vi "Unlock ECU.vi"(8 "error in (no error)":errorcluster, 11 "Node Ptr":T2 format="%.0x") -> (0 "error out":errorcluster)   [LabVIEW 2024, in "Diagnostics Addon System Explorer.lvlib"]
uses:
  Diagnostics Addon System Explorer.lvlib
  Addon Shared/Types/Security.Type.ctl
  <vilib>/NI VeriStand/Custom Device API/Custom Device Item Ref.ctl
  Types/FG.Action.ctl
  Addon Shared/Types/Settings.Channel.ctl
  <vilib>/NI VeriStand/Custom Device API/Custom Device Channel.ctl
  <vilib>/NI VeriStand/Custom Device API/Custom Device Channel Type.ctl
  SubVIs/FileDependency.Create.vi
  Addon Shared/SubVIs/Constants.vi
  <vilib>/NI VeriStand/Custom Device API/NI VeriStand - Get Item Property.vi
  <vilib>/NI VeriStand/Custom Device API/Get Item Property (U32).vi
  <vilib>/NI VeriStand/Custom Device API/Get Item Property (Path).vi
  SubVIs/FileDependency.Get.Target Path.vi
  <vilib>/NI VeriStand/Custom Device API/Get Item Property (Variant).vi
  <vilib>/NI VeriStand/Custom Device API/Get Item Property (String).vi
  <vilib>/NI VeriStand/Custom Device API/Get Item Property (I32).vi
  <vilib>/NI/NI VeriStand Advanced SysDef API/SysDef API/SysDef.Property.Remove.vi
  <vilib>/NI/NI VeriStand Advanced SysDef API/SysDef API/SysDef.Property.Set.vi
  <vilib>/NI/NI VeriStand Advanced SysDef API/_SubVIs/SysDef.Property.Set.Path.vi
  <vilib>/Utility/MD5Checksum.llb/MD5Checksum File.vi
  <vilib>/NI/NI VeriStand Advanced SysDef API/_SubVIs/SysDef.Property.Set.DependentFile.vi
  <vilib>/NI/NI VeriStand Advanced SysDef API/_SubVIs/SysDef.Property.Set.U32.vi
  <vilib>/NI/NI VeriStand Advanced SysDef API/_SubVIs/SysDef.Property.Set.Variant.vi
  <vilib>/NI/NI VeriStand Advanced SysDef API/_SubVIs/SysDef.Property.Set.String.vi
  <vilib>/NI/NI VeriStand Advanced SysDef API/_SubVIs/SysDef.Property.Set.I32.vi
  <vilib>/NI VeriStand/Custom Device Tools/Custom Device Utility Library/NI VeriStand - Search for Item by GUID.vi
  <vilib>/NI VeriStand/Custom Device API/Custom Device API.lvlib
  Addon Shared/Diagnostics Addon Shared.lvlib
  <vilib>/NI VeriStand/Custom Device Tools/Custom Device Utility Library/Custom Device Utility Library.lvlib
panel:
  in  "Host IP Address":string
  in  "Max Key Length":u32
  in  "Optional Parameter":i8 format="%.0x"
  in  "ECU Variant":i8 format="%.0x"
  in  "Access Mode":u32 format="%.0x"
  in  "Seed Key Path":path caption="Seed Key Path (.DLL or .SO)"
  in  "Type":T1
  in  "Master Key":string
  in  "Header":cluster{"Section Name":string}={"Section Name"="Security Settings"}
  in  "SHDocVw.IWebBrowser":refnum<k7>(container)
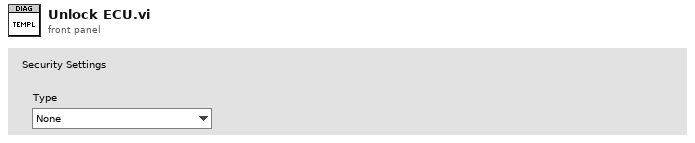
[diagram p1: front panel]
types:
  T1 = typedef "Diagnostics Addon Shared.lvlib/Security.Type.ctl" = enum16{"None", "SeedKey DLL", "MasterKey (Channel)", "MasterKey (Static)", "SeedKey DLL (Windows)"}
  T2 = typedef "Custom Device API.lvlib/Custom Device Item Ref.ctl" = u64
  T3 = typedef "Diagnostics Addon System Explorer.lvlib/FG.Action.ctl" = enum16{"Get", "Set"}
  T4 = typedef "Custom Device API.lvlib/Custom Device Item Info.ctl" = cluster{"Name":string, "Is Channel":bool, "GUID":string, "Is Waveform":bool}
  T5 = typedef "Diagnostics Addon Shared.lvlib/Security.ctl" = cluster{"Type":T1, "Source DLL Path":path, "Target DLL Path":path, "Security Level":u32, "Static Master Key":string, "Max Key Length":u32, "Host IP Address":string, "ECU  Variant":i8, "Optional Parameter":i8}
  T6 = typedef "Custom Device API.lvlib/Custom Device Commands.ctl" = enum16{"Default", "Item renamed", "Shutdown", "Dynamic button pressed"}
  T7 = typedef "Diagnostics Addon Shared.lvlib/Settings.Channel.ctl" = cluster{"Name":string, "Description":string, "Channel":T8}
  T8 = typedef "Custom Device API.lvlib/Custom Device Channel.ctl" = cluster{"Type":T9, "Units":string, "Default Value":dbl, "Faultable":bool, "Scalable":bool}
  T9 = typedef "Custom Device API.lvlib/Custom Device Channel Type.ctl" = enum16{"Input", "Output"}
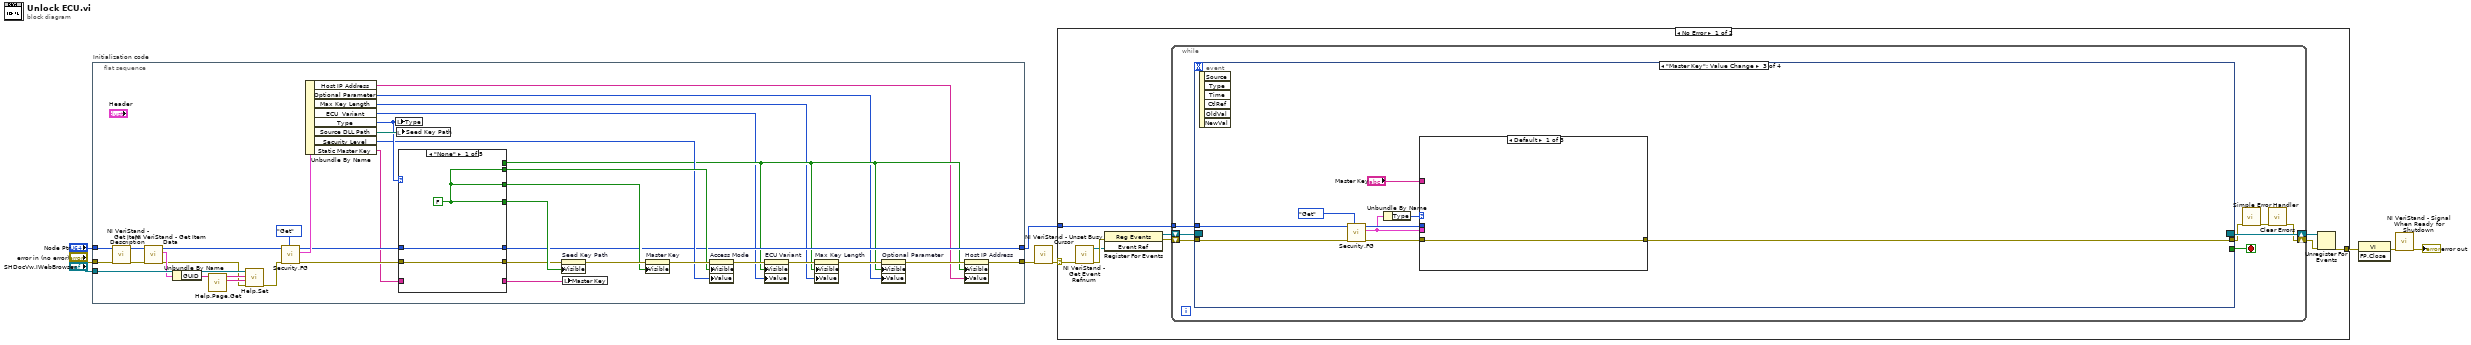
[diagram p0: block diagram]
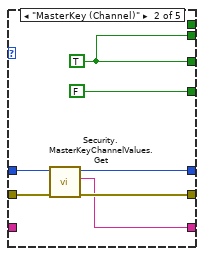
[diagram p2: hidden frame]
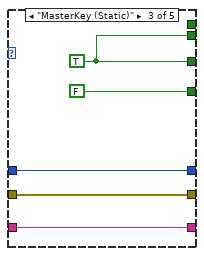
[diagram p3: hidden frame]
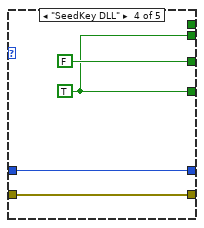
[diagram p4: hidden frame]
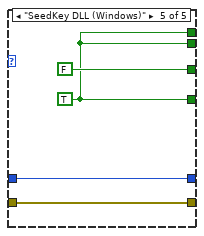
[diagram p5: hidden frame]
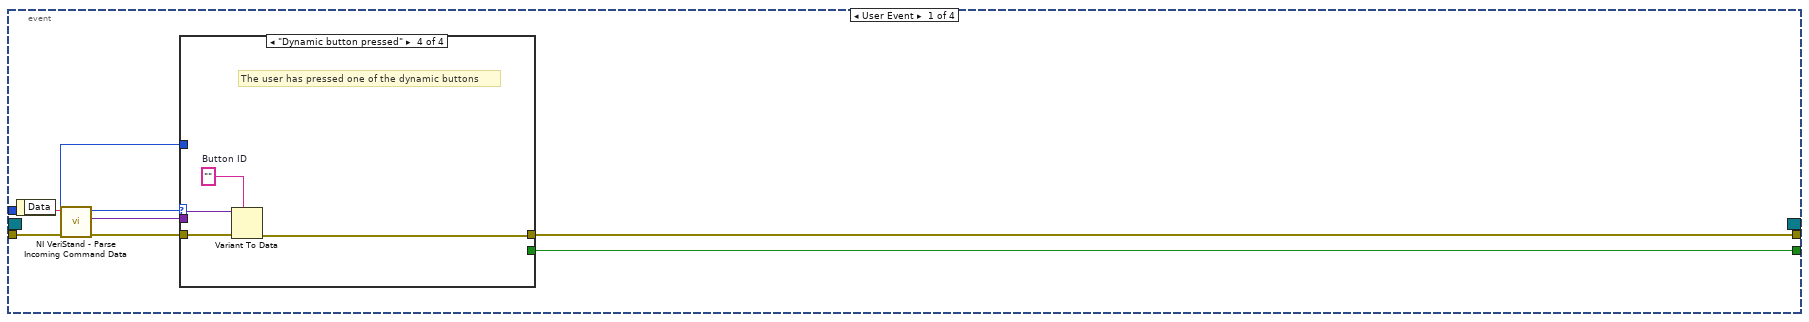
[diagram p6: hidden frame]
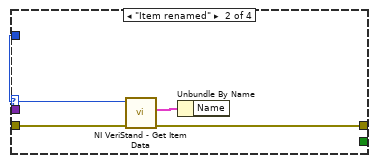
[diagram p8: hidden frame]
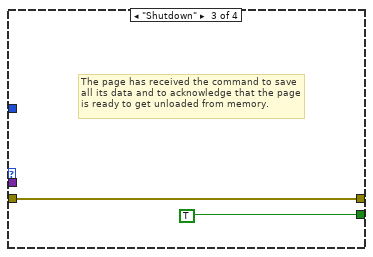
[diagram p9: hidden frame]
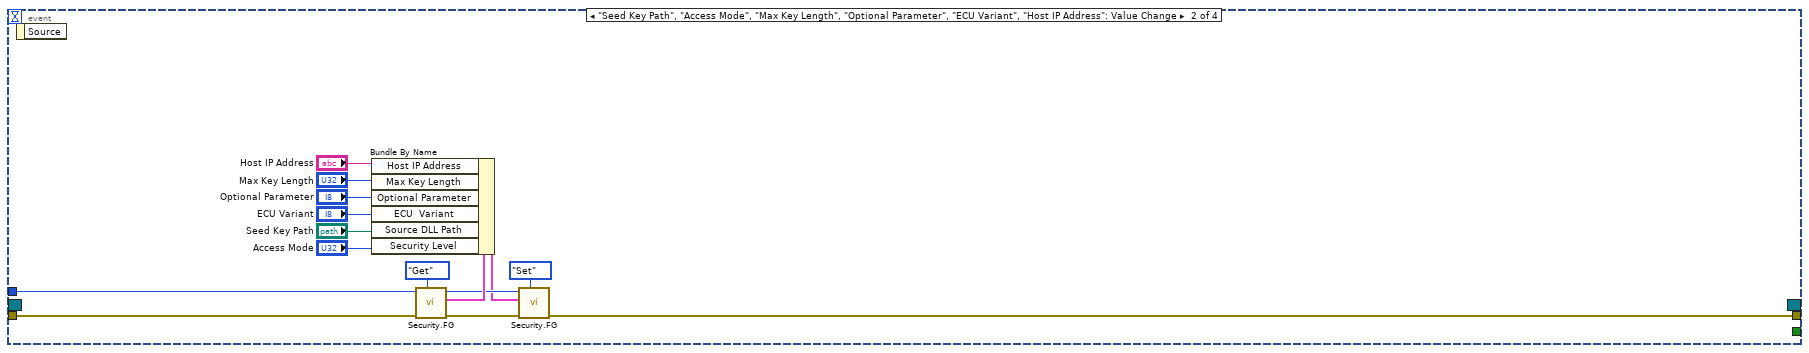
[diagram p10: hidden frame]
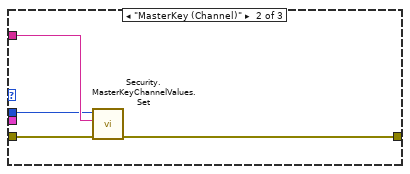
[diagram p11: hidden frame]
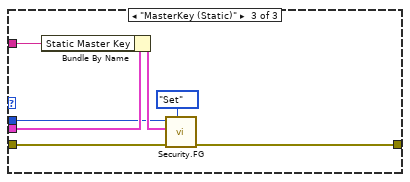
[diagram p12: hidden frame]
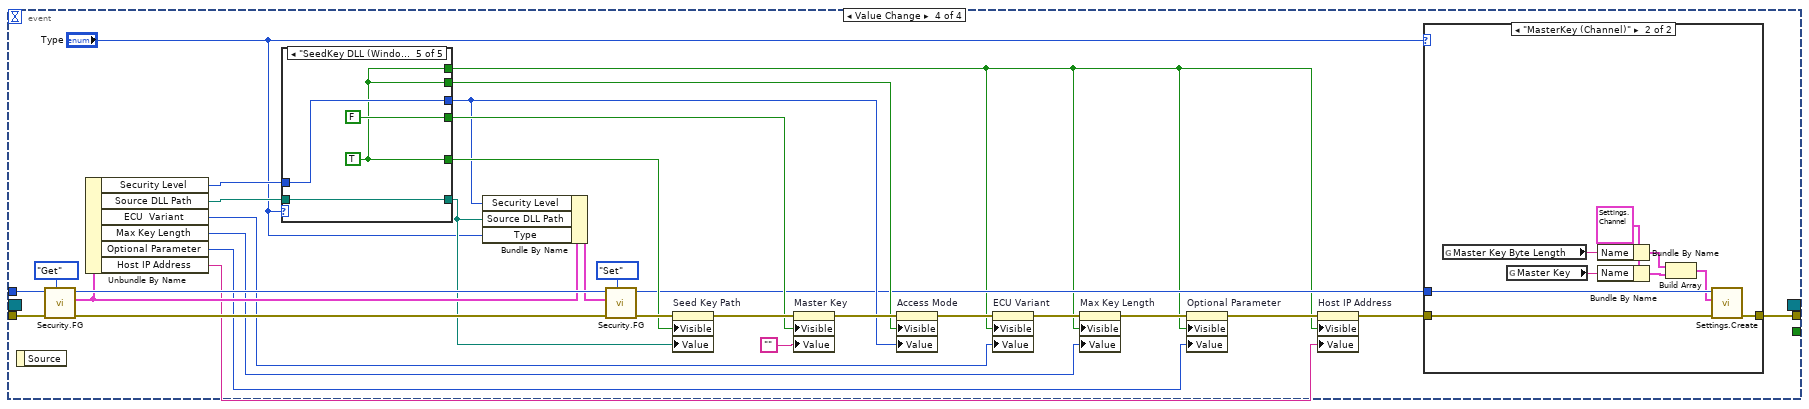
[diagram p13: hidden frame]
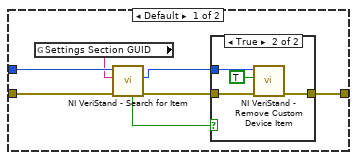
[diagram p14: hidden frame]
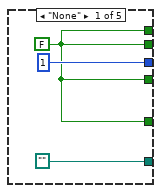
[diagram p16: hidden frame]
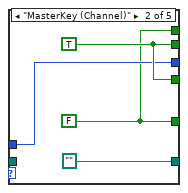
[diagram p17: hidden frame]
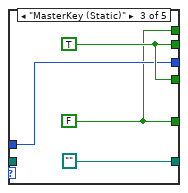
[diagram p18: hidden frame]
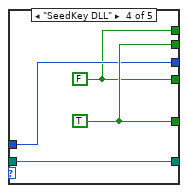
[diagram p19: hidden frame]
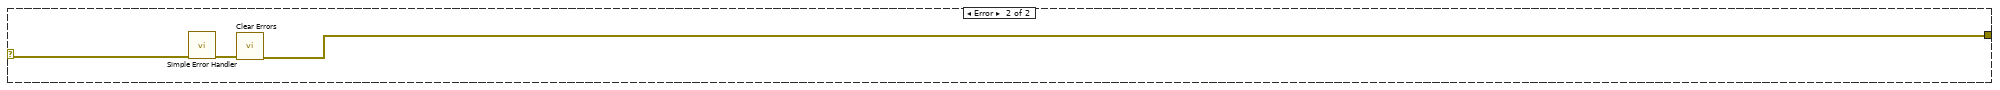
[diagram p20: hidden frame]
diagram:
  n1 = flat-sequence "Initialization code" {
    tunnel: "error in (no error)" -> [w30]
    tunnel: "Node Ptr" -> [w33]
    tunnel: [w15] -> w5
    tunnel: [w22] -> w2
    tunnel: "SHDocVw.IWebBrowser" -> [w45]
    frame #0 {
      n2 = call <vilib>:"NI VeriStand - Get Item Description.vi"("error in (no error)"=w30, "Item Ref in"=w33) -> ("error out"=w46:errorcluster, "Item Ref out"=w47:T2)  [unwired: 8 out]
      n3 = call <vilib>:"NI VeriStand - Get Item Data.vi"("error in (no error)"=w46, "Item Ref in"=w47) -> ("error out"=w27:errorcluster, "Item Info"=w29:T4, "Item Ref out"=w34:T2)  [unwired: 7 out]
      n4 = Unbundle By Name(w29) -> ("GUID"=w28:string)
      n5 = call "Help.Page.Get.vi"("GUID"=w28) -> ("HTML File"=w31:string, "Main CHM File"=w32:string)  [unwired: 9 in]
      n6 = call "Help.Set.vi"("error in (no error)"=w27, "HTML File"=w31, "Main CHM File"=w32, "SHDocVw.IWebBrowser2"=w45) -> ("error out"=w26:errorcluster)  [unwired: 7 in]
      n7 = call "Security.FG.vi"("Action"=FG.Action."Get", "error in (no error)"=w26, "Device Item Ref in"=w34) -> ("error out"=w24:errorcluster, "Security"=w44:T5, "Device Item Ref out"=w25:T2)  [unwired: 6 in]
      n8 = Unbundle By Name(w44) -> ("Host IP Address"=w10:string, "Optional Parameter"=w11:i8, "Max Key Length"=w12:u32, "ECU  Variant"=w13:i8, "Type"=w40:T1, "Source DLL Path"=w42:path, "Security Level"=w35:u32, "Static Master Key"=w20:string)
      n9 = local write "Type"(w40) -> ()
      n10 = local write "Seed Key Path"(w42) -> ()
      n11 = case shown="\"None\"" w40 {
        tunnel: [w50 FALSE FALSE w65 w67] -> w39
        tunnel: [w50 w56 w61 FALSE FALSE] -> w38
        tunnel: [w50 w56 w61 w65 w67] -> w36
        tunnel: w25 -> [w48 w54 w58 w63 w68]
        tunnel: w24 -> [w49 w55 w59 w64 w69]
        tunnel: [w49 w53 w59 w64 w69] -> w23
        tunnel: [w48 w52 w58 w63 w68] -> w22
        tunnel: [_ w51 w60 _ _] -> w21
        tunnel: w20 -> [_ _ w60 _ _]
        tunnel: [_ _ _ _ w67] -> w14
        frame "None" {
          w50 = FALSE
        }
        frame "MasterKey (Channel)" {
          w56 = TRUE
          n12 = call "Security.MasterKeyChannelValues.Get.vi"("error in (no error)"=w55, "Device Item Ref in"=w54) -> ("error out"=w53:errorcluster, "MasterKey"=w51:string, "Section Ref out"=w52:T2)  [unwired: 7 in]
        }
        frame "MasterKey (Static)" {
          w61 = TRUE
        }
        frame "SeedKey DLL" {
          w65 = TRUE
        }
        frame "SeedKey DLL (Windows)" {
          w67 = TRUE
        }
      }
      n13 = property on="Seed Key Path" class="Path"(error in=w23, "Visible"=w39) -> (error out=w41:errorcluster)  [unwired: 1 in, 1 out]
      n14 = local write "Master Key"(w21) -> ()
      n15 = property on="Master Key" class="Str"(error in=w41, "Visible"=w38) -> (error out=w37:errorcluster)  [unwired: 1 in, 1 out]
      n16 = property on="Access Mode" class="DigNum (strict)"(error in=w37, "Visible"=w36, "Value"=w35) -> (error out=w16:errorcluster)  [unwired: 1 in, 1 out]
      n17 = property on="ECU Variant" class="DigNum (strict)"(error in=w16, "Visible"=w14, "Value"=w13) -> (error out=w19:errorcluster)  [unwired: 1 in, 1 out]
      n18 = property on="Max Key Length" class="DigNum (strict)"(error in=w19, "Visible"=w14, "Value"=w12) -> (error out=w18:errorcluster)  [unwired: 1 in, 1 out]
      n19 = property on="Optional Parameter" class="DigNum (strict)"(error in=w18, "Visible"=w14, "Value"=w11) -> (error out=w17:errorcluster)  [unwired: 1 in, 1 out]
      n20 = property on="Host IP Address" class="Str"(error in=w17, "Visible"=w14, "Value"=w10) -> (error out=w15:errorcluster)  [unwired: 1 in, 1 out]
    }
  }
  n21 = call <vilib>:"NI VeriStand - Unset Busy Cursor.vi"("error in (no error)"=w5) -> ("error out"=w4:errorcluster)  [unwired: 10 out]
  n22 = case shown="No Error" w4 {
    selector: w4 -> [w71 w217]
    tunnel: [w76 w215] -> w9
    tunnel: w2 -> [w72 _]
    frame No Error {
      n23 = call <vilib>:"NI VeriStand - Get Event Refnum.vi"("error in (no error)"=w71) -> ("error out"=w79:errorcluster, "Event Ref"=w75:refnum<user-event>)  [unwired: 9 out]
      n24 = register-events(error in=w79, w75) -> (reference out=w73:refnum<event-registration>, error out=w74:errorcluster)  [unwired: 1 in]
      n25 = while {
        tunnel: w72 -> [w83]
        shift-right: [w80] -> w77
        shift-left: w74 -> [w86]
        shift-right: [w87] -> w78
        shift-left: w73 -> [w85]
        stop <- w84 stop-if-true
        n26 = event shown="[2] \"Master Key\": Value Change" {
          selector: w85 -> [_ _ _ _]
          dyn-events: [_ _ _ _] -> w87
          timeout: _ -> [_ _ _ _]
          tunnel: w86 -> [w95 w121 w130 w174]
          tunnel: [w91 _ _ _] -> w84
          tunnel: [w90 w111 w127 w157] -> w82
          tunnel: w83 -> [w89 w120 w129 w173]
          event User Event {
            n27 = event-data() -> ("Data"=w94:string)  [unwired: 1 out]
            n28 = call <vilib>:"NI VeriStand - Parse Incoming Command Data.vi"("error in (no error)"=w95, "Incoming data"=w94) -> ("error out"=w93:errorcluster, "Outgoing data"=w88:variant, "Action"=w92:T6)  [unwired: 7 out]
            n29 = case shown="\"Dynamic button pressed\"" w92 {
              tunnel: w93 -> [w96 w100 w101 w106]
              tunnel: [_ _ TRUE _] -> w91
              tunnel: [w96 w97 w101 w103] -> w90
              tunnel: w89 -> [_ w99 _ _]
              tunnel: w88 -> [_ _ _ w105]
              frame "Default", Default {
              }
              frame "Item renamed" {
                n30 = call <vilib>:"NI VeriStand - Get Item Data.vi"("error in (no error)"=w100, "Item Ref in"=w99) -> ("error out"=w97:errorcluster, "Item Info"=w98:T4)  [unwired: 8 out]
                n31 = Unbundle By Name(w98) -> ()  [unwired: 1 out]
              }
              frame "Shutdown" {
                # "The page has received the command to save all its data and to acknowledge that the page is ready to get unloaded from memory."
              }
              frame "Dynamic button pressed" {
                w104 = ""  # Button ID
                # "The user has pressed one of the dynamic buttons"
                n32 = Variant To Data(error in=w106, type=w104, Variant=w105) -> (error out=w103:errorcluster)  [unwired: 1 out]
              }
            }
          }
          event "Seed Key Path", "Access Mode", "Max Key Length", "Optional Parameter", "ECU Variant", "Host IP Address": Value Change {
            n33 = event-data() -> ()  [unwired: 2 out]
            n34 = call "Security.FG.vi"("Action"=FG.Action."Get", "error in (no error)"=w121, "Device Item Ref in"=w120) -> ("error out"=w117:errorcluster, "Security"=w119:T5, "Device Item Ref out"=w116:T2)  [unwired: 6 in]
            n35 = Bundle By Name(cluster=w119, "Host IP Address"="Host IP Address", "Max Key Length"="Max Key Length", "Optional Parameter"="Optional Parameter", "ECU  Variant"="ECU Variant", "Source DLL Path"="Seed Key Path", "Security Level"="Access Mode") -> (w112:T5)
            n36 = call "Security.FG.vi"("Action"=FG.Action."Set", "error in (no error)"=w117, "Security"=w112, "Device Item Ref in"=w116) -> ("error out"=w111:errorcluster)  [unwired: 5 in, 2 out]
          }
          event "Master Key": Value Change {
            n37 = event-data() -> ()  [unwired: 7 out]
            n38 = call "Security.FG.vi"("Action"=FG.Action."Get", "error in (no error)"=w130, "Device Item Ref in"=w129) -> ("error out"=w126:errorcluster, "Security"=w122:T5, "Device Item Ref out"=w125:T2)  [unwired: 6 in]
            n39 = Unbundle By Name(w122) -> ("Type"=w123:T1)
            n40 = case shown="Default" w123 {
              tunnel: [w131 w134 w139] -> w127
              tunnel: w126 -> [w131 w135 w140]
              tunnel: "Master Key" -> [_ w133 w136]
              tunnel: w125 -> [_ w132 w137]
              tunnel: w122 -> [_ _ w138]
              frame Default {
              }
              frame "MasterKey (Channel)" {
                n41 = call "Security.MasterKeyChannelValues.Set.vi"("error in (no error)"=w135, "Master Key"=w133, "Device Item Ref in"=w132) -> ("error out"=w134:errorcluster)  [unwired: 7 in, 1 out]
              }
              frame "MasterKey (Static)" {
                n42 = Bundle By Name(cluster=w138, "Static Master Key"=w136) -> (w141:T5)
                n43 = call "Security.FG.vi"("Action"=FG.Action."Set", "error in (no error)"=w140, "Security"=w141, "Device Item Ref in"=w137) -> ("error out"=w139:errorcluster)  [unwired: 5 in, 2 out]
              }
            }
          }
          event Value Change {
            n44 = event-data() -> ()  [unwired: 2 out]
            n45 = call "Security.FG.vi"("Action"=FG.Action."Get", "error in (no error)"=w174, "Device Item Ref in"=w173) -> ("error out"=w171:errorcluster, "Security"=w163:T5, "Device Item Ref out"=w170:T2)  [unwired: 6 in]
            n46 = Unbundle By Name(w163) -> ("Security Level"=w158:u32, "Source DLL Path"=w162:path, "ECU  Variant"=w149:i8, "Max Key Length"=w148:u32, "Optional Parameter"=w147:i8, "Host IP Address"=w143:string)
            n47 = case shown="\"SeedKey DLL (Windows)\"" "Type" {
              tunnel: [w196 w199 w203 w209 w211] -> w165
              tunnel: [w196 w201 w205 w207 FALSE] -> w164
              tunnel: w162 -> [_ _ _ w210 w213]
              tunnel: [path "" path "" path "" w210 w213] -> w161
              tunnel: [w196 w201 w205 w209 w211] -> w159
              tunnel: w158 -> [_ w200 w204 w208 w212]
              tunnel: [u32 1 w200 w204 w208 w212] -> w156
              tunnel: [w196 w199 w203 w207 w211] -> w144
              frame "None" {
                w196 = FALSE
              }
              frame "MasterKey (Channel)" {
                w201 = TRUE
                w199 = FALSE
              }
              frame "MasterKey (Static)" {
                w205 = TRUE
                w203 = FALSE
              }
              frame "SeedKey DLL" {
                w207 = FALSE
                w209 = TRUE
              }
              frame "SeedKey DLL (Windows)" {
                w211 = TRUE
              }
            }
            n48 = Bundle By Name(cluster=w163, "Security Level"=w156, "Source DLL Path"=w161, "Type"="Type") -> (w168:T5)
            n49 = call "Security.FG.vi"("Action"=FG.Action."Set", "error in (no error)"=w171, "Security"=w168, "Device Item Ref in"=w170) -> ("error out"=w166:errorcluster, "Device Item Ref out"=w154:T2)  [unwired: 5 in, 1 out]
            n50 = property on="Seed Key Path" class="Path"(error in=w166, "Visible"=w165, "Value"=w161) -> (error out=w167:errorcluster)  [unwired: 1 in, 1 out]
            n51 = property on="Master Key" class="Str"(error in=w167, "Visible"=w164, "Value"="") -> (error out=w160:errorcluster)  [unwired: 1 in, 1 out]
            n52 = property on="Access Mode" class="DigNum (strict)"(error in=w160, "Visible"=w159, "Value"=w156) -> (error out=w152:errorcluster)  [unwired: 1 in, 1 out]
            n53 = property on="ECU Variant" class="DigNum (strict)"(error in=w152, "Visible"=w144, "Value"=w149) -> (error out=w151:errorcluster)  [unwired: 1 in, 1 out]
            n54 = property on="Max Key Length" class="DigNum (strict)"(error in=w151, "Visible"=w144, "Value"=w148) -> (error out=w150:errorcluster)  [unwired: 1 in, 1 out]
            n55 = property on="Optional Parameter" class="DigNum (strict)"(error in=w150, "Visible"=w144, "Value"=w147) -> (error out=w146:errorcluster)  [unwired: 1 in, 1 out]
            n56 = property on="Host IP Address" class="Str"(error in=w146, "Visible"=w144, "Value"=w143) -> (error out=w145:errorcluster)  [unwired: 1 in, 1 out]
            n57 = case shown="\"MasterKey (Channel)\"" "Type" {
              tunnel: w145 -> [w179 w195]
              tunnel: [w180 w194] -> w157
              tunnel: w154 -> [w181 w193]
              frame Default {
                n58 = global read "Constants.vi" "Settings Section GUID"() -> (w176:string)
                n59 = call-poly <vilib>:"NI VeriStand - Search for Item.vi"("error in"=w179, "Item GUID"=w176, "Section Ref in"=w181) -> ("error out"=w178:errorcluster, "Item Ref"=w177:T2, "Found"=w175:bool)  [unwired: 5 in, 1 out]
                n60 = case shown="True" w175 {
                  tunnel: [w182 w186] -> w180
                  tunnel: w178 -> [w182 w185]
                  tunnel: w177 -> [_ w184]
                  frame False {
                  }
                  frame True {
                    n61 = call <vilib>:"NI VeriStand - Remove Custom Device Item.vi"("error in (no error)"=w185, "Force Delete (F)"=TRUE, "Item Ref in"=w184) -> ("error out"=w186:errorcluster)  [unwired: 7 in, 1 out]
                  }
                }
              }
              frame "MasterKey (Channel)" {
                w187 = T7 {"Name"="Byte Length", "Description"="", "Channel"={"Type"=enum."Input", "Units"="", "Default Value"=0.0, "Faultable"=FALSE, "Scalable"=FALSE}} ("cluster")
                n62 = global read "Constants.vi" "Master Key Byte Length"() -> (w189:string)
                n63 = global read "Constants.vi" "Master Key"() -> (w188:string)
                n64 = Bundle By Name(cluster=w187, "Name"=w189) -> (w190:T7)
                n65 = Bundle By Name(cluster=w187, "Name"=w188) -> (w192:T7)
                n66 = Build Array(w190, w192) -> (w191:T7[])
                n67 = call "Settings.Create.vi"("error in (no error)"=w195, "Settings Channels"=w191, "Section Ref in"=w193) -> ("error out"=w194:errorcluster)  [unwired: 7 in, 1 out]
              }
            }
          }
        }
        n68 = call <vilib>:"Simple Error Handler.vi"("error in (no error)"=w82) -> ("error out"=w81:errorcluster)  [unwired: 1 in, 7 out]
        n69 = call <vilib>:"Clear Errors.vi"("error in (no error)"=w81) -> ("error out"=w80:errorcluster)  [unwired: 1 in, 5 out]
      }
      n70 = Unregister For Events(event registration refnum=w78, error in=w77) -> (error out=w76:errorcluster)
    }
    frame Error {
      n71 = call <vilib>:"Simple Error Handler.vi"("error in (no error)"=w217) -> ("error out"=w216:errorcluster)  [unwired: 1 in, 7 out]
      n72 = call <vilib>:"Clear Errors.vi"("error in (no error)"=w216) -> ("error out"=w215:errorcluster)  [unwired: 1 in, 5 out]
    }
  }
  n73 = invoke class="VI" method="FP.Close"(error in=w9) -> (error out=w8:errorcluster)  [unwired: 2 in, 2 out]
  n74 = call <vilib>:"NI VeriStand - Signal When Ready for Shutdown.vi"("error in (no error)"=w8) -> ("error out"=→"error out":errorcluster)  [unwired: 10 out]
